vi "Query.vi"(5 "buffered":bool=TRUE, 6 "commandTimeout":i32=-1, 7 "CommandType":i32(ring)=-1 items=["Text"=1, "StoredProcedure"=4, "TableDirect"=512], 8 "error in (no error)":errorcluster, 9 "DynamicParameters":refnum<class "DynamicParameters.lvclass">, 10 "sql":string, 11 "PGJDPMapper in":refnum<class "Mapper.lvclass">) -> (0 "error out":errorcluster, 2 "Query Result out":refnum<class "Query Result.lvclass">, 3 "PGJDPMapper out":refnum<class "Mapper.lvclass">)   [LabVIEW 2020, in "ORM_sqlite_jdp.lvlib" / "Mapper.lvclass"]
uses:
  Mapper.lvclass
  C:/Program Files/National Instruments/LabVIEW 2020/vi.lib/Viviota/shared/ORM.lvlibp/SqlMapper/SqlMapper.lvclass
  <vilib>/Viviota/shared/ORM.lvlibp/Query Result/Query Result.lvclass
  <vilib>/Viviota/shared/ORM.lvlibp/DynamicParameters/DynamicParameters.lvclass
  dbc/DBC.lvclass
  PGJDPParameter/Parameter.lvclass
  C:/Program Files/National Instruments/LabVIEW 2020/vi.lib/Viviota/shared/ORM.lvlibp/DynamicParameters/DynamicParameters.lvclass
  <vilib>/drjdpowell/SQLite Library/SQL Statement/SQL Statement.lvclass/SQL Statement.ctl
  <vilib>/drjdpowell/SQLite Library/SQL Statement/Next Bind (name).vi
  <vilib>/drjdpowell/SQLite Library/SQL Statement/Next Bind.vi
  <vilib>/drjdpowell/SQLite Library/SQL Statement/Step.vi
  PGJDPResult/Result.lvclass
  C:/Program Files/National Instruments/LabVIEW 2020/vi.lib/Viviota/shared/ORM.lvlibp/Query Result/Query Result.lvclass
  <vilib>/Viviota/shared/ORM.lvlibp/SqlMapper/Read DbConnection.vi
  dbc/Read Connection.vi
  <vilib>/Viviota/shared/ORM.lvlibp/DynamicParameters/Read ParameterNames.vi
  <vilib>/Viviota/shared/ORM.lvlibp/DynamicParameters/Read ParameterValues.vi
  <vilib>/drjdpowell/SQLite Library/SQL Statement/Bind Parameters.vi
  <vilib>/drjdpowell/SQLite Library/SQL Statement/Error Message.vi
  <vilib>/Viviota/shared/ORM.lvlibp/DbConnection/DbConnection.lvclass
  <vilib>/drjdpowell/SQLite Library/SQL Connection/Connection.lvclass
  <vilib>/drjdpowell/SQLite Library/SQL Statement/SQL Statement.lvclass
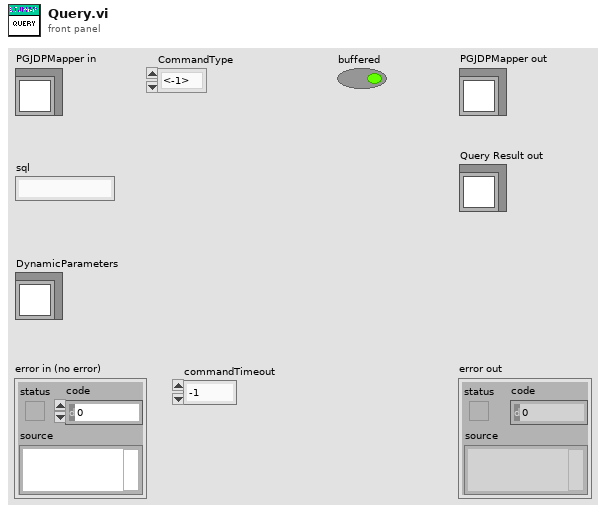
[diagram p1: front panel]
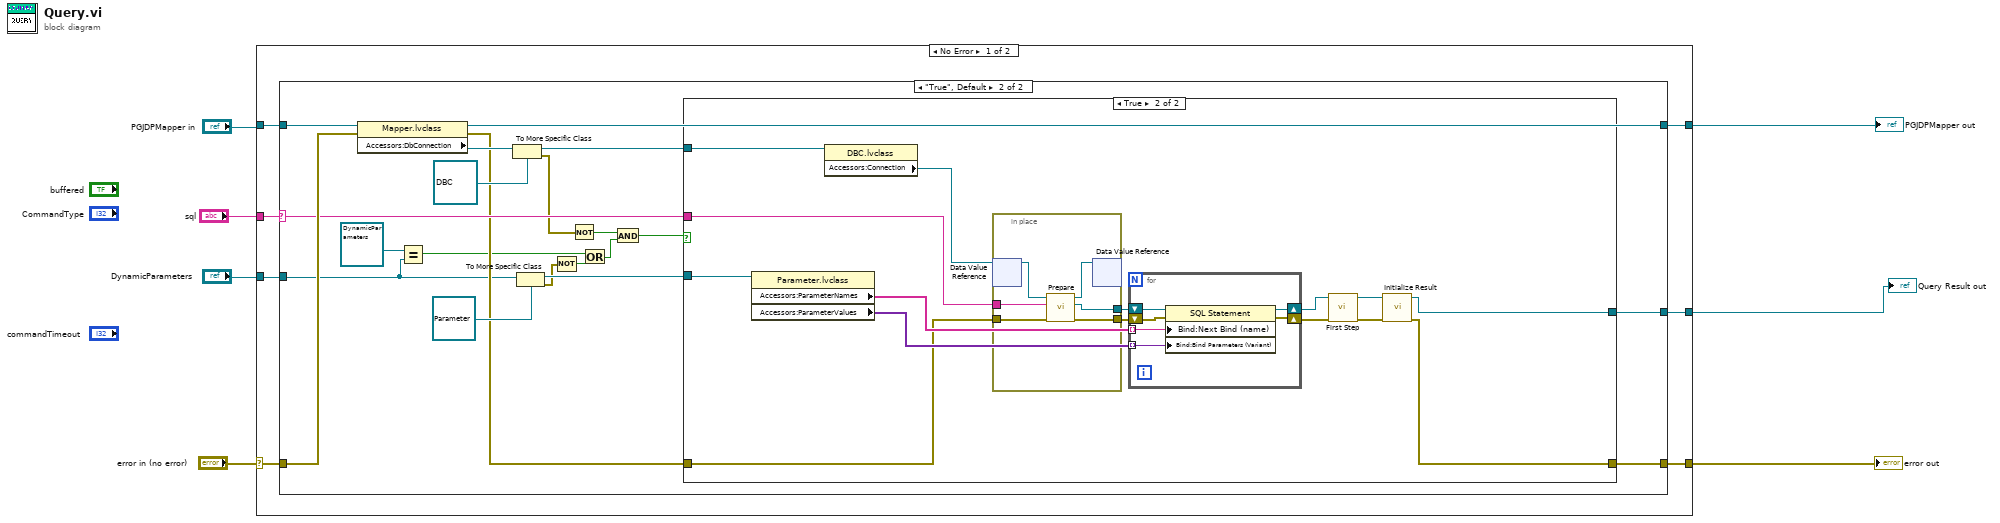
[diagram p0: block diagram]
diagram:
  n1 = case shown="No Error" "error in (no error)" {
    selector: "error in (no error)" -> [w12 w67]
    tunnel: "PGJDPMapper in" -> [w14 w66]
    tunnel: [w13 w66] -> w6
    tunnel: [w11 w67] -> w2
    tunnel: "sql" -> [w10 _]
    tunnel: "DynamicParameters" -> [w9 _]
    tunnel: [w8 _] -> w1
    frame No Error {
      n2 = case shown="\"True\", Default" w10 {
        selector: w10 -> [_ w30]
        tunnel: w14 -> [w16 w37]
        tunnel: [w16 w36] -> w13
        tunnel: w12 -> [w15 w35]
        tunnel: [w15 w27] -> w11
        tunnel: w9 -> [_ w18]
        tunnel: [_ w26] -> w8
        frame "" {
        }
        frame "True", Default {
          n3 = property class="Mapper.lvclass"(reference=w37, error in=w35) -> (reference out=w36:refnum<class "Mapper.lvclass">, error out=w28:errorcluster, "Accessors:DbConnection"=w34:refnum<class "DbConnection.lvclass">)
          n4 = Equal?(x=refnum<class "DynamicParameters.lvclass"> refnum ("DynamicParameters"), y=w18) -> (x = y?=w23:bool)
          n5 = To More Specific Class(target class=refnum<class "DBC.lvclass"> refnum ("ORM_pgsql_jdp.lvlib:DBC.lvclass"), reference=w34) -> (specific class reference=w29:refnum<class "DBC.lvclass">, error out=w20:errorcluster)  [unwired: 1 in]
          n6 = To More Specific Class(target class=refnum<class "Parameter.lvclass"> refnum ("ORM_pgsql_jdp.lvlib:PGJDPParameter.lvclass"), reference=w18) -> (specific class reference=w31:refnum<class "Parameter.lvclass">, error out=w19:errorcluster)  [unwired: 1 in]
          n7 = Not(x=w19) -> (.not. x?=w24:bool)
          n8 = Not(x=w20) -> (.not. x?=w21:bool)
          n9 = Or(x=w23, y=w24) -> (x .or. y?=w22:bool)
          n10 = And(x=w21, y=w22) -> (x .and. y?=w17:bool)
          n11 = case shown="True" w17 {
            tunnel: w31 -> [_ w45]
            tunnel: w30 -> [_ w44]
            tunnel: w29 -> [_ w46]
            tunnel: w28 -> [w38 w43]
            tunnel: [w38 w39] -> w27
            tunnel: [_ w40] -> w26
            frame False {
            }
            frame True {
              n12 = property class="Parameter.lvclass"(reference=w45) -> ("Accessors:ParameterNames"=w51:string[], "Accessors:ParameterValues"=w50:variant[])  [unwired: 1 in, 2 out]
              n13 = property class="DBC.lvclass"(reference=w46) -> ("Accessors:Connection"=w47:refnum<data-value>)  [unwired: 1 in, 2 out]
              n14 = in-place {
                in-place-border: w43 -> [w59]
                in-place-border: w44 -> [w58]
                in-place-border: [w57] -> w53
                in-place-border: [w56] -> w52
                n15 = in-place-dvr #1(w47) -> (w55:refnum<class "Connection.lvclass">)  [unwired: 1 out]
                n16 = call <vilib>:"Prepare.vi"("error in (no error)"=w59, "SQL"=w58, "SQLite Connection in"=w55) -> ("error out"=w57:errorcluster, "SQL Statement"=w56:refnum<class "SQL Statement.lvclass">, "SQLite Connection"=w54:refnum<class "Connection.lvclass">)  [unwired: 4 in, 2 out]
                n17 = in-place-dvr #1(w54) -> ()  [unwired: 2 out]
              }
              n18 = for {
                tunnel: w51 -> [w63] mode=indexing
                tunnel: w50 -> [w62] mode=indexing
                shift-right: [w61] -> w49
                shift-left: w52 -> [w64]
                shift-right: [w60] -> w48
                shift-left: w53 -> [w65]
                n19 = property class="SQL Statement"(reference=w64, error in=w65, "Bind:Next Bind (name)"=w63, "Bind:Bind Parameters (Variant)"=w62) -> (reference out=w61:refnum<class "SQL Statement.lvclass">, error out=w60:errorcluster)
              }
              n20 = call <vilib>:"First Step.vi"("error in (no error)"=w48, "SQL Statement in"=w49) -> ("error out"=w41:errorcluster, "SQL Statement"=w42:refnum<class "SQL Statement.lvclass">)  [unwired: 7 in, 1 out]
              n21 = call "Initialize Result.vi"("error in (no error)"=w41, "SQL Statement"=w42) -> ("error out"=w39:errorcluster, "PGJDPResult out"=w40:refnum<class "Result.lvclass">)  [unwired: 8 in]
            }
          }
        }
      }
    }
    frame Error {
    }
  }
  "error out" <- w2
  "PGJDPMapper out" <- w6
  "Query Result out" <- w1
